vi "Mock Circulation Loop met sub-Vi.vi"() -> ()   [LabVIEW 2024]
uses:
  <vilib>/DAQmx/write.llb/DAQmx Write (Digital 1D Bool NChan 1Samp 1Line).vi
  <vilib>/DAQmx/miscellaneous.llb/DAQmx Fill In Error Info.vi
  <vilib>/Utility/file.llb/Write Delimited Spreadsheet (string).vi
  <vilib>/Utility/file.llb/Write Delimited Spreadsheet (DBL).vi
  <vilib>/DAQmx/create/channels.llb/DAQmx Create Channel (AO-Voltage-Basic).vi
  <vilib>/DAQmx/create/channels.llb/DAQmx Create Channel (AI-Voltage-Basic).vi
  <vilib>/DAQmx/write.llb/DAQmx Write (Analog DBL 1Chan 1Samp).vi
  <vilib>/DAQmx/read.llb/DAQmx Read (Analog 1D DBL NChan 1Samp).vi
  <vilib>/DAQmx/create/channels.llb/DAQmx Create Channel (DO-Digital Output).vi
panel:
  in  "Set pressure Hybrid Heart (Bar)":dbl
  in  "Analog output pressure regulator":tag="Dev1/ao0"
  out "Actual Press. from Regulator (Bar)":dbl=0.5073311185231432
  out "Flow sensors":cluster{dbl[], dbl[]}[](graph)=[{[0.014721000000463391], [-6.750071131370961, -6.750071131370961, -6.750071131370961, -6.750071131370961, -6.750071131370961, -6.750071131370961, -6.750071131370961, -6.750071131370961, -6.750071131370961, -6.750071131370961, -6.750071131370961, -6.750071131370961, -6.750071131370961, -6.750071131370961, -6.750071131370961, -6.750071131370961, -6.755156296628295, -6.755156296628295, -6.750071131370961, -6.750071131370961, -6.750071131370961, -6.750071131370961, -6.750071131370961, -6.750071131370961, -6.750071131370961, -6.750071131370961, -6.750071131370961, -6.755156296628295, -6.750071131370961, -6.750071131370961, -6.750071131370961, -6.750071131370961, -6.750071131370961, -6.750071131370961, -6.750071131370961, -6.750071131370961, -6.750071131370961, -6.750071131370961, -6.750071131370961, -6.750071131370961, -6.750071131370961, -6.750071131370961, -6.750071131370961, -6.750071131370961, -6.750071131370961, -6.750071131370961, -6.750071131370961, -6.750071131370961, -6.750071131370961, -6.750071131370961, -6.750071131370961, -6.750071131370961, -6.750071131370961, -6.750071131370961, -6.750071131370961, -6.750071131370961, -6.750071131370961, -6.750071131370961, -6.750071131370961, -6.750071131370961, -6.750071131370961, -6.750071131370961, -6.750071131370961, -6.750071131370961, -6.750071131370961, -6.750071131370961, -6.750071131370961, -6.750071131370961, -6.750071131370961, -6.750071131370961, -6.755156296628295, -6.750071131370961, -6.750071131370961, -6.750071131370961, -6.750071131370961, -6.750071131370961, -6.755156296628295, -6.750071131370961, -6.750071131370961, -6.750071131370961, -6.750071131370961, -6.750071131370961, -6.750071131370961, -6.750071131370961, -6.750071131370961, -6.750071131370961, -6.750071131370961, -6.750071131370961, -6.750071131370961, -6.750071131370961, -6.750071131370961, -6.750071131370961, -6.750071131370961, -6.755156296628295, -6.744985966113629, -6.750071131370961, -6.750071131370961, -6.750071131370961, -6.750071131370961, -6.750071131370961, -6.750071131370961, -6.750071131370961, -6.750071131370961, -6.750071131370961, -6.750071131370961, -6.750071131370961, -6.750071131370961, -6.750071131370961, -6.755156296628295, -6.750071131370961, -6.750071131370961, -6.750071131370961, -6.750071131370961, -6.755156296628295, -6.750071131370961, -6.750071131370961, -6.750071131370961, -6.750071131370961, -6.750071131370961, -6.750071131370961, -6.755156296628295, -6.750071131370961, -6.750071131370961, -6.750071131370961, -6.750071131370961, -6.750071131370961, -6.750071131370961, -6.750071131370961, -6.750071131370961, -6.750071131370961, -6.750071131370961, -6.755156296628295, -6.750071131370961, -6.750071131370961, -6.750071131370961, -6.750071131370961, -6.750071131370961, -6.750071131370961, -6.750071131370961, -6.750071131370961, -6.750071131370961, -6.750071131370961, -6.750071131370961, -6.750071131370961, -6.750071131370961, -6.750071131370961, -6.755156296628295, -6.750071131370961, -6.750071131370961, -6.750071131370961, -6.750071131370961, -6.750071131370961, -6.750071131370961, -6.750071131370961, -6.750071131370961, -6.750071131370961, -6.750071131370961, -6.750071131370961, -6.750071131370961, -6.750071131370961, -6.750071131370961, -6.750071131370961, -6.750071131370961, -6.750071131370961, -6.750071131370961, -6.750071131370961, -6.750071131370961, -6.750071131370961, -6.744985966113629, -6.750071131370961, -6.750071131370961, -6.750071131370961, -6.750071131370961, -6.750071131370961, -6.750071131370961, -6.750071131370961, -6.750071131370961, -6.750071131370961, -6.750071131370961, -6.750071131370961, -6.750071131370961, -6.750071131370961, -6.750071131370961, -6.750071131370961, -6.750071131370961, -6.750071131370961, -6.750071131370961, -6.750071131370961, -6.750071131370961, -6.755156296628295, -6.755156296628295, -6.750071131370961, -6.750071131370961, -6.750071131370961, -6.750071131370961, -6.750071131370961, -6.750071131370961, -6.750071131370961, -6.744985966113629, -6.750071131370961, -6.750071131370961, -6.750071131370961, -6.750071131370961, -6.750071131370961, -6.750071131370961, -6.750071131370961, -6.750071131370961, -6.750071131370961, -6.750071131370961, -6.750071131370961, -6.750071131370961, -6.750071131370961, -6.750071131370961, -6.755156296628295, -6.750071131370961, -6.750071131370961, -6.750071131370961, -6.750071131370961, -6.750071131370961, -6.755156296628295, -6.750071131370961, -6.750071131370961, -6.750071131370961, -6.750071131370961, -6.750071131370961, -6.750071131370961, -6.750071131370961, -6.750071131370961, -6.750071131370961, -6.750071131370961, -6.750071131370961, -6.750071131370961, -6.750071131370961, -6.750071131370961, -6.750071131370961, -6.750071131370961, -6.750071131370961, -6.750071131370961, -6.750071131370961, -6.750071131370961, -6.750071131370961, -6.750071131370961, -6.750071131370961, -6.750071131370961, -6.750071131370961, -6.750071131370961, -6.750071131370961, -6.750071131370961, -6.750071131370961, -6.750071131370961, -6.750071131370961, -6.750071131370961, -6.750071131370961, -6.755156296628295, -6.750071131370961, -6.750071131370961, -6.750071131370961, -6.755156296628295, -6.750071131370961, -6.750071131370961, -6.750071131370961, -6.750071131370961, -6.750071131370961, -6.750071131370961, -6.755156296628295, -6.750071131370961, -6.750071131370961, -6.750071131370961, -6.750071131370961, -6.750071131370961, -6.750071131370961, -6.750071131370961, -6.750071131370961, -6.750071131370961, -6.750071131370961, -6.750071131370961, -6.750071131370961, -6.750071131370961, -6.750071131370961, -6.750071131370961, -6.750071131370961, -6.750071131370961, -6.750071131370961, -6.750071131370961, -6.750071131370961, -6.750071131370961, -6.750071131370961, -6.750071131370961, -6.750071131370961, -6.750071131370961, -6.755156296628295, -6.750071131370961, -6.750071131370961, -6.750071131370961, -6.750071131370961, -6.750071131370961, -6.750071131370961, -6.750071131370961, -6.750071131370961, -6.755156296628295, -6.750071131370961, -6.750071131370961, -6.750071131370961, -6.750071131370961, -6.755156296628295, -6.750071131370961, -6.755156296628295, -6.750071131370961, -6.750071131370961, -6.750071131370961, -6.750071131370961, -6.750071131370961, -6.750071131370961, -6.750071131370961, -6.750071131370961, -6.750071131370961, -6.750071131370961, -6.750071131370961, -6.750071131370961, -6.750071131370961, -6.750071131370961, -6.750071131370961, -6.750071131370961, -6.750071131370961, -6.750071131370961, -6.750071131370961, -6.750071131370961, -6.750071131370961, -6.750071131370961, -6.750071131370961, -6.750071131370961, -6.750071131370961, -6.750071131370961, -6.750071131370961, -6.750071131370961, -6.750071131370961, -6.750071131370961, -6.750071131370961, -6.750071131370961, -6.750071131370961, -6.750071131370961, -6.750071131370961, -6.750071131370961, -6.750071131370961, -6.750071131370961, -6.750071131370961, -6.755156296628295, -6.750071131370961, -6.750071131370961, -6.750071131370961, -6.750071131370961, -6.750071131370961, -6.750071131370961, -6.750071131370961, -6.750071131370961, -6.750071131370961, -6.755156296628295, -6.750071131370961, -6.750071131370961, -6.750071131370961, -6.750071131370961, -6.750071131370961, -6.750071131370961, -6.750071131370961, -6.750071131370961, -6.750071131370961, -6.750071131370961, -6.750071131370961, -6.750071131370961, -6.750071131370961, -6.750071131370961, -6.750071131370961, -6.750071131370961, -6.750071131370961, -6.750071131370961, -6.750071131370961, -6.750071131370961, -6.750071131370961, -6.750071131370961, -6.750071131370961, -6.750071131370961, -6.750071131370961, -6.750071131370961, -6.750071131370961, -6.750071131370961, -6.750071131370961, -6.750071131370961, -6.744985966113629, -6.750071131370961, -6.750071131370961, -6.750071131370961, -6.750071131370961, -6.750071131370961, -6.750071131370961, -6.750071131370961, -6.755156296628295, -6.750071131370961, -6.750071131370961, -6.750071131370961, -6.750071131370961, -6.750071131370961, -6.750071131370961, -6.750071131370961, -6.755156296628295, -6.750071131370961]}, ...(2 in all)]
  in  "Seconds per data point":dbl
  out "Pressure sensors":cluster{dbl[], dbl[]}[](graph)=[{[0.014721000000463391], [-2.2408081975299865, -2.2408081975299865, -2.4339157389476895, -2.2408081975299865, -1.8545931146945804, -2.4339157389476895, -2.2408081975299865, -2.2408081975299865, -2.2408081975299865, -2.2408081975299865, -2.4339157389476895, -2.4339157389476895, -2.4339157389476895, -2.4339157389476895, -2.4339157389476895, -2.2408081975299865, -2.2408081975299865, -2.2408081975299865, -2.4339157389476895, -2.2408081975299865, -2.4339157389476895, -2.2408081975299865, -2.4339157389476895, -2.2408081975299865, -2.2408081975299865, -2.2408081975299865, -2.2408081975299865, -2.2408081975299865, -2.4339157389476895, -2.2408081975299865, -2.4339157389476895, -2.2408081975299865, -2.4339157389476895, -2.4339157389476895, -2.4339157389476895, -2.4339157389476895, -2.4339157389476895, -2.2408081975299865, -2.2408081975299865, -2.2408081975299865, -2.4339157389476895, -2.2408081975299865, -2.4339157389476895, -2.4339157389476895, -2.4339157389476895, -2.2408081975299865, -2.2408081975299865, -2.2408081975299865, -2.4339157389476895, -2.2408081975299865, -2.4339157389476895, -2.4339157389476895, -2.2408081975299865, -2.2408081975299865, -2.4339157389476895, -2.4339157389476895, -2.2408081975299865, -2.2408081975299865, -2.2408081975299865, -2.4339157389476895, -2.4339157389476895, -2.2408081975299865, -2.4339157389476895, -2.4339157389476895, -2.4339157389476895, -2.4339157389476895, -2.4339157389476895, -2.4339157389476895, -2.2408081975299865, -2.2408081975299865, -2.2408081975299865, -2.4339157389476895, -2.2408081975299865, -2.4339157389476895, -2.2408081975299865, -2.2408081975299865, -2.4339157389476895, -2.4339157389476895, -2.4339157389476895, -2.4339157389476895, -2.4339157389476895, -2.4339157389476895, -2.4339157389476895, -2.4339157389476895, -2.4339157389476895, -2.4339157389476895, -2.4339157389476895, -2.2408081975299865, -2.4339157389476895, -2.4339157389476895, -2.2408081975299865, -2.4339157389476895, -2.4339157389476895, -2.2408081975299865, -2.4339157389476895, -2.4339157389476895, -2.4339157389476895, -2.2408081975299865, -2.4339157389476895, -2.4339157389476895, -2.4339157389476895, -2.2408081975299865, -2.4339157389476895, -2.4339157389476895, -2.2408081975299865, -2.2408081975299865, -2.4339157389476895, -2.4339157389476895, -2.2408081975299865, -2.4339157389476895, -2.4339157389476895, -2.0477006561122835, -2.4339157389476895, -2.2408081975299865, -2.4339157389476895, -2.2408081975299865, -2.2408081975299865, -2.4339157389476895, -2.0477006561122835, -2.2408081975299865, -2.2408081975299865, -2.4339157389476895, -2.2408081975299865, -2.4339157389476895, -2.4339157389476895, -2.4339157389476895, -2.4339157389476895, -2.4339157389476895, -2.2408081975299865, -2.0477006561122835, -2.4339157389476895, -2.4339157389476895, -2.4339157389476895, -2.2408081975299865, -2.4339157389476895, -2.4339157389476895, -2.4339157389476895, -2.4339157389476895, -2.2408081975299865, -2.4339157389476895, -2.4339157389476895, -2.4339157389476895, -2.2408081975299865, -2.4339157389476895, -2.4339157389476895, -2.4339157389476895, -2.4339157389476895, -2.4339157389476895, -2.2408081975299865, -2.4339157389476895, -2.4339157389476895, -1.8545931146945804, -2.2408081975299865, -2.4339157389476895, -2.2408081975299865, -2.2408081975299865, -2.4339157389476895, -2.2408081975299865, -2.4339157389476895, -2.0477006561122835, -2.4339157389476895, -2.2408081975299865, -2.0477006561122835, -2.4339157389476895, -2.4339157389476895, -2.2408081975299865, -2.2408081975299865, -2.4339157389476895, -2.2408081975299865, -2.4339157389476895, -2.2408081975299865, -2.4339157389476895, -2.2408081975299865, -2.2408081975299865, -2.4339157389476895, -2.4339157389476895, -2.4339157389476895, -2.0477006561122835, -2.2408081975299865, -2.4339157389476895, -2.2408081975299865, -2.4339157389476895, -2.2408081975299865, -2.4339157389476895, -2.4339157389476895, -2.4339157389476895, -2.4339157389476895, -2.2408081975299865, -2.4339157389476895, -2.4339157389476895, -2.2408081975299865, -2.2408081975299865, -2.4339157389476895, -2.4339157389476895, -2.2408081975299865, -2.4339157389476895, -2.4339157389476895, -2.2408081975299865, -2.2408081975299865, -2.4339157389476895, -2.4339157389476895, -2.2408081975299865, -2.2408081975299865, -2.2408081975299865, -2.2408081975299865, -2.2408081975299865, -2.4339157389476895, -2.4339157389476895, -2.4339157389476895, -2.2408081975299865, -2.4339157389476895, -2.2408081975299865, -2.4339157389476895, -2.6270232803653926, -2.4339157389476895, -2.2408081975299865, -2.2408081975299865, -2.2408081975299865, -2.4339157389476895, -2.4339157389476895, -2.2408081975299865, -2.4339157389476895, -2.4339157389476895, -2.2408081975299865, -2.4339157389476895, -2.4339157389476895, -2.4339157389476895, -2.2408081975299865, -2.4339157389476895, -1.8545931146945804, -2.4339157389476895, -2.4339157389476895, -2.4339157389476895, -2.4339157389476895, -2.4339157389476895, -2.0477006561122835, -2.4339157389476895, -2.4339157389476895, -2.2408081975299865, -2.4339157389476895, -2.2408081975299865, -2.4339157389476895, -2.4339157389476895, -2.4339157389476895, -2.2408081975299865, -2.2408081975299865, -1.8545931146945804, -2.4339157389476895, -2.4339157389476895, -2.2408081975299865, -2.4339157389476895, -2.4339157389476895, -2.4339157389476895, -2.4339157389476895, -2.4339157389476895, -2.4339157389476895, -2.4339157389476895, -2.2408081975299865, -2.2408081975299865, -2.4339157389476895, -2.4339157389476895, -2.4339157389476895, -2.2408081975299865, -2.4339157389476895, -2.4339157389476895, -2.4339157389476895, -2.4339157389476895, -2.4339157389476895, -2.4339157389476895, -2.4339157389476895, -2.4339157389476895, -2.4339157389476895, -2.4339157389476895, -2.2408081975299865, -2.4339157389476895, -2.4339157389476895, -2.2408081975299865, -2.4339157389476895, -2.2408081975299865, -2.2408081975299865, -2.4339157389476895, -2.4339157389476895, -2.2408081975299865, -2.4339157389476895, -2.4339157389476895, -2.4339157389476895, -2.2408081975299865, -2.4339157389476895, -2.2408081975299865, -2.4339157389476895, -2.2408081975299865, -2.4339157389476895, -2.4339157389476895, -2.2408081975299865, -2.2408081975299865, -2.4339157389476895, -2.4339157389476895, -1.8545931146945804, -2.4339157389476895, -2.2408081975299865, -2.2408081975299865, -2.4339157389476895, -2.4339157389476895, -2.2408081975299865, -2.4339157389476895, -2.2408081975299865, -2.4339157389476895, -2.2408081975299865, -2.4339157389476895, -2.2408081975299865, -2.2408081975299865, -2.2408081975299865, -2.2408081975299865, -2.2408081975299865, -2.2408081975299865, -2.4339157389476895, -2.2408081975299865, -2.4339157389476895, -2.4339157389476895, -2.4339157389476895, -2.2408081975299865, -2.4339157389476895, -2.4339157389476895, -2.4339157389476895, -2.2408081975299865, -2.2408081975299865, -2.2408081975299865, -2.4339157389476895, -2.2408081975299865, -2.4339157389476895, -2.4339157389476895, -2.4339157389476895, -2.2408081975299865, -2.4339157389476895, -2.4339157389476895, -2.2408081975299865, -2.4339157389476895, -2.4339157389476895, -2.4339157389476895, -2.2408081975299865, -2.4339157389476895, -2.4339157389476895, -2.2408081975299865, -2.4339157389476895, -2.0477006561122835, -2.4339157389476895, -2.4339157389476895, -2.4339157389476895, -2.2408081975299865, -2.4339157389476895, -2.4339157389476895, -2.2408081975299865, -2.4339157389476895, -2.4339157389476895, -2.2408081975299865, -2.4339157389476895, -2.2408081975299865, -2.4339157389476895, -2.4339157389476895, -2.4339157389476895, -2.2408081975299865, -2.4339157389476895, -2.4339157389476895, -2.4339157389476895, -2.2408081975299865, -2.4339157389476895, -2.4339157389476895, -2.4339157389476895, -2.2408081975299865, -2.4339157389476895, -2.2408081975299865, -2.4339157389476895, -2.4339157389476895, -2.4339157389476895, -2.2408081975299865, -1.8545931146945804, -2.4339157389476895, -2.2408081975299865, -2.4339157389476895, -2.4339157389476895, -2.2408081975299865, -2.2408081975299865, -2.4339157389476895, -2.2408081975299865, -2.4339157389476895, -2.4339157389476895, -2.2408081975299865, -2.4339157389476895, -2.2408081975299865, -2.2408081975299865, -2.4339157389476895, -2.2408081975299865, -2.2408081975299865, -2.2408081975299865, -2.4339157389476895, -2.4339157389476895, -2.4339157389476895, -2.4339157389476895, -2.2408081975299865, -2.4339157389476895, -2.2408081975299865, -2.4339157389476895, -2.4339157389476895, -2.2408081975299865, -2.2408081975299865]}, ...(2 in all)]
  out "Elapsed time":dbl=0.014721000000463391
  in  "Input port all sensors":tag="Dev1/ai3:7"
  in  "Start/Stop solenoid valves":bool
  in  "Closed time (ms)":dbl=700.0
  in  "Open time (ms)":dbl=300.0
  in  "STOP":bool
  in  "line grouping":i32(ring) items=["one channel for each line", "one channel for all lines"]
  in  "Port input Solenoid valve":tag="Dev1/port0/line0:1"
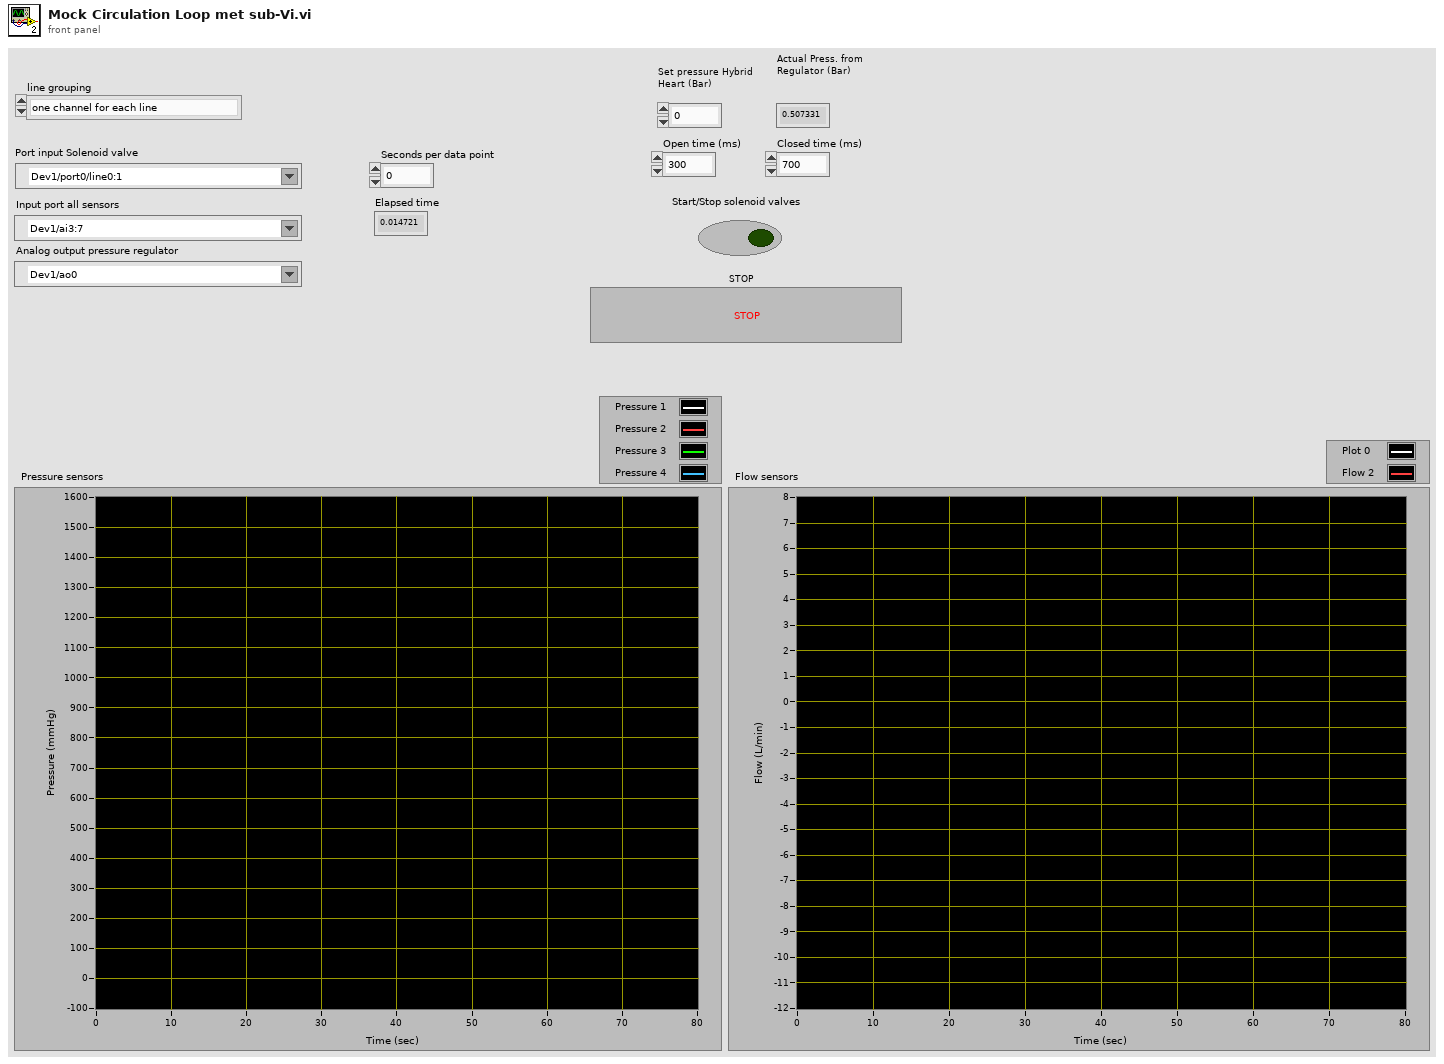
[diagram p1: front panel]
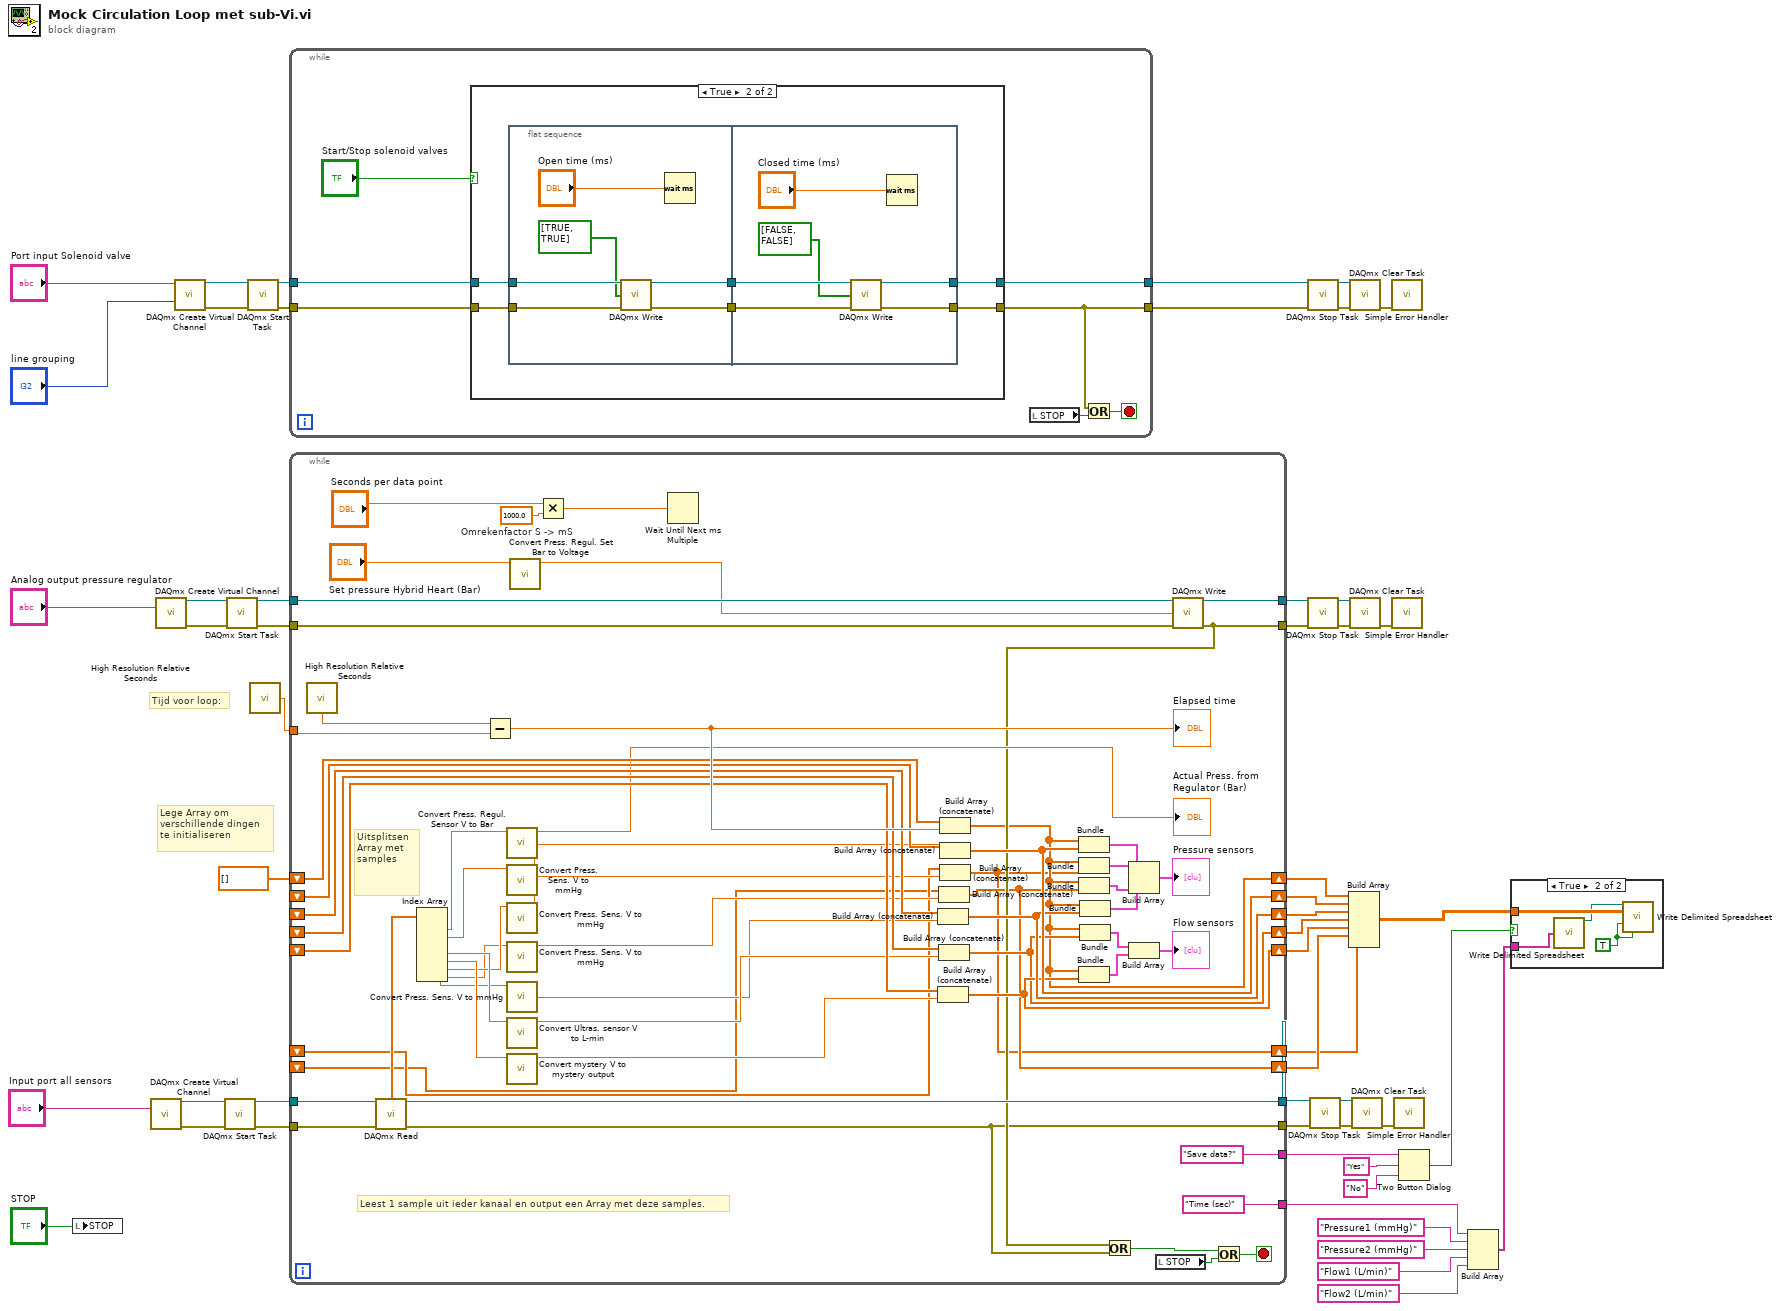
[diagram p0: block diagram]
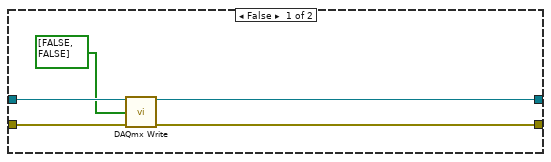
[diagram p3: hidden frame]
diagram:
  # "Tijd voor loop:"
  # "Lege Array om\nverschillende dingen \nte initialiseren"
  n1 = local write "STOP"("STOP") -> ()
  n2 = call-poly <vilib>:"DAQmx Create Virtual Channel.vi"("physical channels"="Input port all sensors") -> ("task out"=w38:refnum<k21>, "error out"=w37:errorcluster)  [unwired: 13 in]
  n3 = call-poly <vilib>:"DAQmx Create Virtual Channel.vi"("physical channels"="Analog output pressure regulator") -> ("task out"=w29:refnum<k21>, "error out"=w28:errorcluster)  [unwired: 13 in]
  n4 = call-poly <vilib>:"DAQmx Create Virtual Channel.vi"("lines"="Port input Solenoid valve", "line grouping"="line grouping") -> ("task out"=w50:refnum<k21>, "error out"=w51:errorcluster)  [unwired: 12 in]
  n5 = call <vilib>:"DAQmx Start Task.vi"("task/channels in"=w38, "error in"=w37) -> ("task out"=w36:refnum<k21>, "error out"=w35:errorcluster)  [unwired: 12 in]
  n6 = call <vilib>:"DAQmx Start Task.vi"("task/channels in"=w29, "error in"=w28) -> ("task out"=w25:refnum<k21>, "error out"=w26:errorcluster)  [unwired: 12 in]
  n7 = call <vilib>:"DAQmx Start Task.vi"("task/channels in"=w50, "error in"=w51) -> ("task out"=w48:refnum<k21>, "error out"=w47:errorcluster)  [unwired: 12 in]
  n8 = call <vilib>:"High Resolution Relative Seconds.vi"() -> ("relative seconds"=w40:dbl)
  n9 = while {
    tunnel: w48 -> [w58]
    tunnel: w47 -> [w57]
    tunnel: [w54] -> w45
    tunnel: [w56] -> w44
    stop <- w55 stop-if-true
    n10 = case shown="True" "Start/Stop solenoid valves" {
      tunnel: w58 -> [w64 w68]
      tunnel: w57 -> [w63 w67]
      tunnel: [w61 w66] -> w54
      tunnel: [w60 w65] -> w56
      frame False {
        n11 = call-poly <vilib>:"DAQmx Write.vi"("task/channels in"=w64, "data"=bool[] [FALSE, FALSE], "error in"=w63) -> ("task out"=w60:refnum<k21>, "error out"=w61:errorcluster)  [unwired: 10 in, 1 out]
      }
      frame True {
        n12 = flat-sequence {
          tunnel: w68 -> [w76]
          tunnel: w67 -> [w75]
          tunnel: [w73] -> w70
          tunnel: [w72] -> w69
          tunnel: w70 -> [w81]
          tunnel: w69 -> [w80]
          tunnel: [w79] -> w65
          tunnel: [w78] -> w66
          frame #0 {
            n13 = call-poly <vilib>:"DAQmx Write.vi"("task/channels in"=w76, "data"=bool[] [TRUE, TRUE], "error in"=w75) -> ("task out"=w73:refnum<k21>, "error out"=w72:errorcluster)  [unwired: 10 in, 1 out]
            n14 = Wait (ms)(milliseconds to wait="Open time (ms)") -> ()  [unwired: 1 out]
          }
          frame #1 {
            n15 = call-poly <vilib>:"DAQmx Write.vi"("task/channels in"=w81, "data"=bool[] [FALSE, FALSE], "error in"=w80) -> ("task out"=w79:refnum<k21>, "error out"=w78:errorcluster)  [unwired: 10 in, 1 out]
            n16 = Wait (ms)(milliseconds to wait="Closed time (ms)") -> ()  [unwired: 1 out]
          }
        }
      }
    }
    n17 = local read "STOP"() -> (w53:bool)
    n18 = Or(x=w54, y=w53) -> (x .or. y?=w55:bool)
  }
  n19 = while {
    tunnel: w36 -> [w140]
    tunnel: w35 -> [w139]
    tunnel: w40 -> [w134]
    shift-right: [w93] -> w19
    shift-left: dbl[] [] -> [w132]
    shift-right: [w128] -> w18
    shift-left: _ -> [w130]
    shift-right: [w127] -> w17
    shift-left: _ -> [w129]
    tunnel: [w123] -> w34
    tunnel: [w96] -> w33
    shift-right: [w119] -> w16
    shift-left: _ -> [w122]
    shift-right: [w120] -> w15
    shift-left: _ -> [w121]
    tunnel: w26 -> [w95]
    tunnel: w25 -> [w115]
    tunnel: [w97] -> w21
    tunnel: [w114] -> w20
    tunnel: ["Time (sec)"] -> w8
    tunnel: ["Save data?" ("message")] -> w4
    shift-right: [w88] -> w2
    shift-left: _ -> [w85]
    shift-right: [w87] -> w1
    shift-left: _ -> [w86]
    stop <- w106 stop-if-true
    w136 = 1000.0  # Omrekenfactor S -> mS
    # "Leest 1 sample uit ieder kanaal en output een Array met deze samples."
    # "Uitsplitsen Array met \nsamples"
    n20 = call <vilib>:"High Resolution Relative Seconds.vi"() -> ("relative seconds"=w135:dbl)
    n21 = call-poly <vilib>:"DAQmx Read.vi"("task/channels in"=w140, "error in"=w139) -> ("task out"=w123:refnum<k21>, "data"=w131:dbl[], "error out"=w96:errorcluster)  [unwired: 11 in]
    n22 = Index Array(array=w131) -> (element #1=w113:dbl, element #2=w100:dbl, element #3=w99:dbl, element #4=w102:dbl, element #5=w101:dbl, element #6=w90:dbl, element #7=w89:dbl)  [unwired: 7 in]
    n23 = Subtract(x=w135, y=w134) -> (x-y=w133:dbl)
    "Elapsed time" <- w133
    n24 = call "Convert Press. Regul. Sensor V to Bar.vi"("V. Regulator Press. Sensor"=w113) -> ("Press. at Regulator (Bar)"=→"Actual Press. from Regulator (Bar)":dbl)  [unwired: 10 in]
    n25 = call "Convert Press. Sens. V to mmHg.vi"("Waveform"=w100) -> ("Numeric"=w94:dbl)  [unwired: 10 in]
    n26 = call "Convert Press. Sens. V to mmHg.vi"("Waveform"=w90) -> ("Numeric"=w92:dbl)  [unwired: 10 in]
    n27 = call "Convert Press. Sens. V to mmHg.vi"("Waveform"=w89) -> ("Numeric"=w91:dbl)  [unwired: 10 in]
    n28 = call "Convert Press. Sens. V to mmHg.vi"("Waveform"=w99) -> ("Numeric"=w98:dbl)  [unwired: 10 in]
    n29 = call "Convert Ultras. sensor V to L-min.vi"("Waveform"=w102) -> ("Numeric"=w104:dbl)  [unwired: 10 in]
    n30 = call "Convert mystery V to mystery output.vi"("Waveform"=w101) -> ("Numeric"=w103:dbl)  [unwired: 10 in]
    n31 = call "Convert Press. Regul. Set Bar to Voltage.vi"("Set pressure Hybrid Heart (Bar)"="Set pressure Hybrid Heart (Bar)") -> ("Numeric"=w110:dbl)  [unwired: 10 in]
    n32 = Multiply(x="Seconds per data point", y=w136) -> (x*y=w138:dbl)
    n33 = Wait Until Next ms Multiple(millisecond multiple=w138) -> ()  [unwired: 1 out]
    n34 = Build Array (concatenate)(w129, w98) -> (w127:dbl[])
    n35 = Build Array (concatenate)(w121, w103) -> (w120:dbl[])
    n36 = Build Array (concatenate)(w85, w91) -> (w88:dbl[])
    n37 = Build Array (concatenate)(w122, w104) -> (w119:dbl[])
    n38 = Build Array (concatenate)(w132, w133) -> (w93:dbl[])
    n39 = Build Array (concatenate)(w130, w94) -> (w128:dbl[])
    n40 = Build Array (concatenate)(w86, w92) -> (w87:dbl[])
    n41 = Bundle(w93, w128) -> (w126:cluster{dbl[], dbl[]})  [unwired: 1 in]
    n42 = Bundle(w93, w87) -> (w84:cluster{dbl[], dbl[]})  [unwired: 1 in]
    n43 = Bundle(w93, w88) -> (w83:cluster{dbl[], dbl[]})  [unwired: 1 in]
    n44 = Bundle(w93, w120) -> (w117:cluster{dbl[], dbl[]})  [unwired: 1 in]
    n45 = Bundle(w93, w127) -> (w125:cluster{dbl[], dbl[]})  [unwired: 1 in]
    n46 = Bundle(w93, w119) -> (w118:cluster{dbl[], dbl[]})  [unwired: 1 in]
    n47 = Build Array(w84, w126, w125, w83) -> (→"Pressure sensors":cluster{dbl[], dbl[]}[])
    n48 = Build Array(w118, w117) -> (→"Flow sensors":cluster{dbl[], dbl[]}[])
    n49 = local read "STOP"() -> (w105:bool)
    n50 = call-poly <vilib>:"DAQmx Write.vi"("task/channels in"=w115, "data"=w110, "error in"=w95) -> ("task out"=w114:refnum<k21>, "error out"=w97:errorcluster)  [unwired: 10 in, 1 out]
    n51 = Or(x=w97, y=w96) -> (x .or. y?=w107:bool)
    n52 = Or(x=w107, y=w105) -> (x .or. y?=w106:bool)
  }
  n53 = call <vilib>:"DAQmx Stop Task.vi"("task/channels in"=w44, "error in"=w45) -> ("task out"=w43:refnum<k21>, "error out"=w42:errorcluster)  [unwired: 12 in]
  n54 = call <vilib>:"DAQmx Stop Task.vi"("task/channels in"=w20, "error in"=w21) -> ("task out"=w23:refnum<k21>, "error out"=w24:errorcluster)  [unwired: 12 in]
  n55 = call <vilib>:"DAQmx Stop Task.vi"("task/channels in"=w34, "error in"=w33) -> ("task out"=w31:refnum<k21>, "error out"=w32:errorcluster)  [unwired: 12 in]
  n56 = Build Array(w19, w18, w17, w16, w15, w2, w1) -> (w14:dbl[][])
  n57 = call <vilib>:"DAQmx Clear Task.vi"("task in"=w43, "error in"=w42) -> ("error out"=w46:errorcluster)  [unwired: 13 in]
  n58 = call <vilib>:"DAQmx Clear Task.vi"("task in"=w23, "error in"=w24) -> ("error out"=w22:errorcluster)  [unwired: 13 in]
  n59 = call <vilib>:"DAQmx Clear Task.vi"("task in"=w31, "error in"=w32) -> ("error out"=w30:errorcluster)  [unwired: 13 in]
  n60 = call <vilib>:"Simple Error Handler.vi"("error in (no error)"=w46) -> ()  [unwired: 4 in, 5 out]
  n61 = call <vilib>:"Simple Error Handler.vi"("error in (no error)"=w22) -> ()  [unwired: 4 in, 5 out]
  n62 = call <vilib>:"Simple Error Handler.vi"("error in (no error)"=w30) -> ()  [unwired: 4 in, 5 out]
  n63 = Two Button Dialog(message=w4, 1:"No" ("F button name (\"Cancel\")"), 2:"Yes" ("T button name (\"OK\")")) -> (T button?=w7:bool)
  n64 = Build Array(w8, "Pressure1 (mmHg)", "Pressure2 (mmHg)", "Flow1 (L/min)", "Flow2 (L/min)") -> (w9:string[])
  n65 = case shown="True" w7 {
    tunnel: w14 -> [_ w144]
    tunnel: w9 -> [_ w143]
    frame False {
    }
    frame True {
      w141 = TRUE ("transpose? (no:F)")
      n66 = call-poly <vilib>:"Write Delimited Spreadsheet.vi"("1D data"=w143) -> ("new file path (Not A Path if cancelled)"=w142:path)  [unwired: 13 in, 1 out]
      n67 = call-poly <vilib>:"Write Delimited Spreadsheet.vi"("file path (dialog if empty)"=w142, "2D data"=w144, "append to file? (new file:F)"=w141, "transpose? (no:F)"=w141) -> ()  [unwired: 10 in, 2 out]
    }
  }
